vi "Check Type.vi"(11 "Buffer Configuration":T1) -> (3 "Type":T4)   [LabVIEW 2021, in "CIF_CIPC_Chn.lvclass"]
uses:
  CIF_CIPC_Chn.lvclass
  <vilib>/Utility/Data Type/Type Definitions/Data Type.ctl
  Typedef/Buffer Configuration Data.ctl
  <vilib>/CIF Foundation/CIF CIPC/TypeDefs/Backpressure References.ctl
  <vilib>/CIF Foundation/CIF CIPC/TypeDefs/Backpressure Names.ctl
  <vilib>/CIF Foundation/CIF CIPC/SubVIs/Decode Array Element Data.vi
  <vilib>/Utility/error.llb/Trim Whitespace.vi
  CIF_CIPC_Chn.lvclass/CIF_CIPC_Chn.ctl
  <vilib>/CIF Foundation/CIF CIPC/CIF_NI_CIPC.lvlib
  <vilib>/Utility/Data Type/NI_Data Type.lvlib
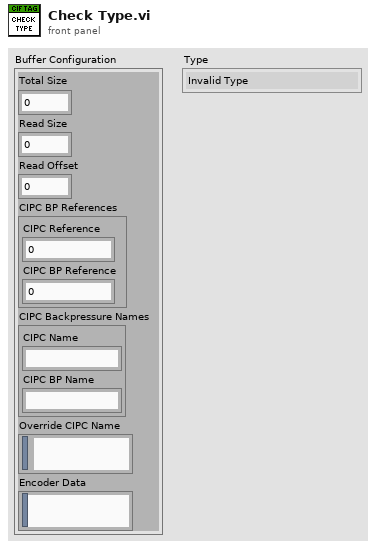
[diagram p1: front panel]
types:
  T1 = typedef "CIF_CIPC_Chn.lvclass/Buffer Configuration Data.ctl" = cluster{"Total Size":u32, "Read Size":u32, "Read Offset":u32, "CIPC BP References":T2, "CIPC Backpressure Names":T3, "Override CIPC Name":string, "Encoder Data":string}
  T2 = typedef "CIF_NI_CIPC.lvlib/Backpressure References.ctl" = cluster{"CIPC Reference":u64, "CIPC BP Reference":u64}
  T3 = typedef "CIF_NI_CIPC.lvlib/Backpressure Names.ctl" = cluster{"CIPC Name":string, "CIPC BP Name":string}
  T4 = typedef "NI_Data Type.lvlib/Data Type.ctl" = enum8{"Invalid Type", "Void", "I8", "I16", "I32", "I64", "U8", "U16", "U32", "U64", "Single Float", "Double Float", "Extended Float", "Single Complex", "Double Complex", "Extended Complex", "Enum U8", "Enum U16", "Enum U32", "Enum U64", "Single Float With Unit", "Double Float With Unit", "Extended Float With Unit", "Single Complex with Unit", "Double Complex with Unit", "Extended Complex with Unit", "Boolean", "String", "Path", "Picture", "Tag", "Array", "Cluster", "Variant", "LV Variant", "Waveform", "Timestamp", "Digital Waveform", "Digital Data", "ExpressData", "Refnum", "External Data", "VI", "Poly VI", "LabVIEW Class Instance", "Fixed Point", "Set Collection", "Map Collection"}
  T5 = typedef "CIF_NI_CIPC.lvlib/Data Encoding.ctl" = cluster{"Data Struct Info":cluster{"Alignment":T6, "Endian":T7, "Array Info":T8, "Total Length (bytes)":i32}, "Data Elements":T9[]}
  T6 = typedef "CIF_NI_CIPC.lvlib/Alignment.ctl" = enum16{"Natural", "Packed"}
  T7 = typedef "DataTypes_CIF_U.lvlib/Endian.ctl" = enum16{"Little Endian", "Big Endian"}
  T8 = typedef "CIF_NI_CIPC.lvlib/Data Struct Array Info.ctl" = cluster{"Array":bool, "Array_Size":i32, "Elem_Size":i32, "Prepended Length":bool}
  T9 = typedef "CIF_NI_CIPC.lvlib/Data Element.ctl" = cluster{"Name":string, "Type":T4, "Size":u32, "Offset":u32}
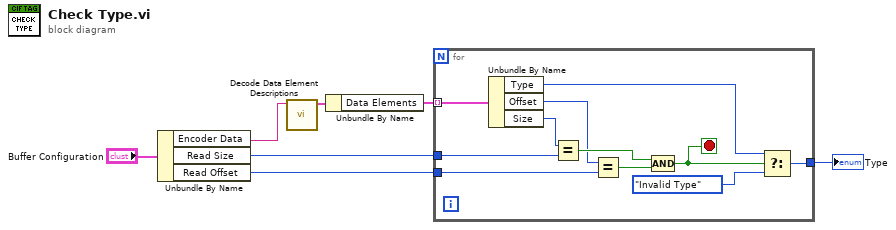
[diagram p0: block diagram]
diagram:
  n1 = Unbundle By Name("Buffer Configuration") -> ("Encoder Data"=w4:string, "Read Size"=w5:u32, "Read Offset"=w6:u32)
  n2 = call <vilib>:"Decode Data Element Descriptions.vi"("Encoder Data Description"=w4) -> ("Data Encoding"=w2:T5)  [unwired: 10 in]
  n3 = Unbundle By Name(w2) -> ("Data Elements"=w1:T9[])
  n4 = for {
    tunnel: w1 -> [w17] mode=indexing
    tunnel: w6 -> [w16]
    tunnel: w5 -> [w15]
    tunnel: [w9] -> w3
    stop <- w8 stop-if-true
    n5 = Unbundle By Name(w17) -> ("Type"=w10:T4, "Offset"=w11:u32, "Size"=w14:u32)
    n6 = Equal?(x=w14, y=w15) -> (x = y?=w13:bool)
    n7 = Equal?(x=w11, y=w16) -> (x = y?=w12:bool)
    n8 = Compound Arithmetic op=AND(w13, w12) -> (w8:bool)
    n9 = Select(t=w10, s=w8, f=Data_Type."Invalid Type") -> (s? t:f=w9:T4)
  }
  "Type" <- w3
